vi "RDC-calculate_length.vi"(11 "Element map":map{dbl, T1}(c390)) -> (2 "L":dbl[](array[numeric]))   [LabVIEW 2020, in "RDC-Reflection_Data_Computation.lvlib"]
doc: "Takes an element map (frequency to data point) and returns an array of lengths L, one per frequency."
uses:
  RDC-Reflection_Data_Computation.lvlib
  Reflector/RFH-common_data_format_element.ctl
  Reflector/RFH-Reflection_File_Handler.lvlib
panel:
  out "Tau":dbl[](array[numeric])
  out "tau":dbl
  out "arctan(x)":dbl
  out "Theta":dbl
  out "l":dbl format="%#_6p"
  out "vp":dbl
  out "Beta":dbl
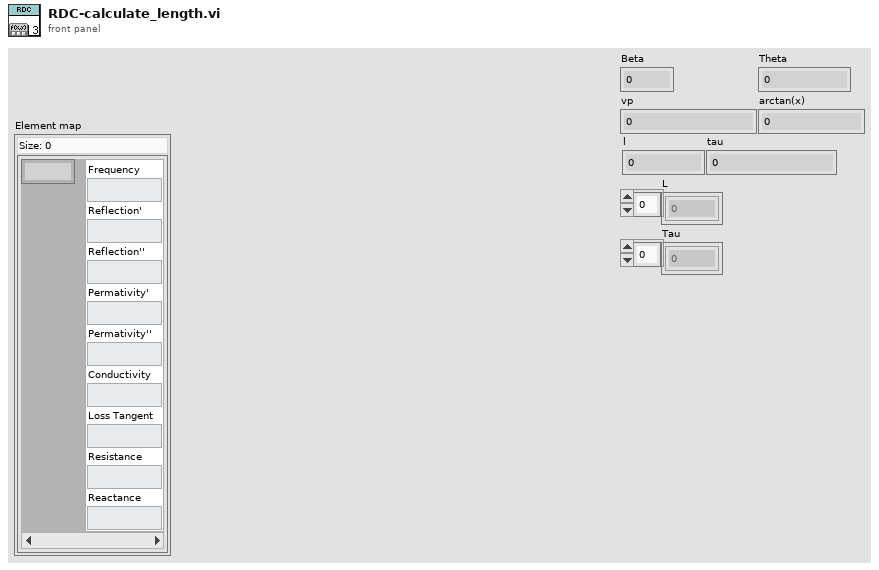
[diagram p1: front panel]
types:
  T1 = typedef "RFH-Reflection_File_Handler.lvlib/RFH-common_data_format_element.ctl" = cluster{"Frequency":dbl, "Reflection'":dbl, "Reflection''":dbl, "Permativity'":dbl, "Permativity''":dbl, "Conductivity":dbl, "Loss Tangent":dbl, "Resistance":dbl, "Reactance":dbl}
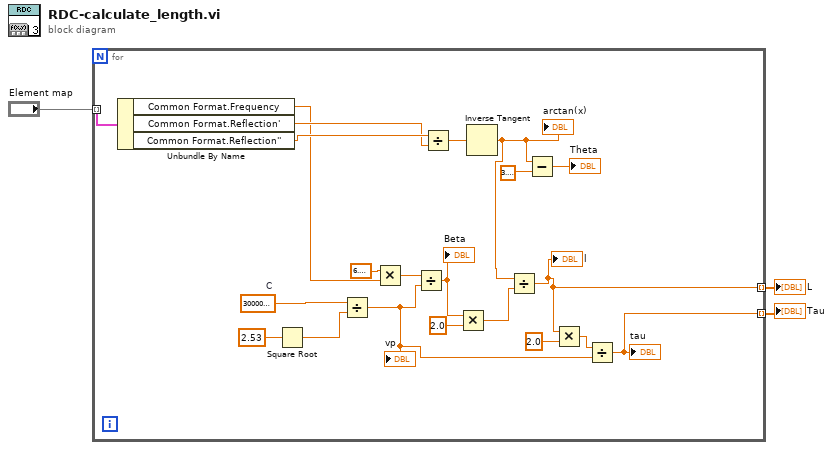
[diagram p0: block diagram]
diagram:
  n1 = for {
    tunnel: "Element map" -> [w24] mode=indexing
    tunnel: [w5] -> w2 mode=indexing
    tunnel: [w4] -> w1 mode=indexing
    w23 = 300000000.0  # C
    n2 = Unbundle By Name(w24) -> ("Common Format.Frequency"=w6:dbl, "Common Format.Reflection'"=w7:dbl, "Common Format.Reflection''"=w8:dbl)
    n3 = Square Root(x=2.53) -> (sqrt(x)=w21:dbl)
    n4 = Divide(x=w23, y=w21) -> (x/y=w9:dbl)
    "vp" <- w9
    n5 = Multiply(x=6.283185307179586, y=w6) -> (x*y=w19:dbl)
    n6 = Divide(x=w19, y=w9) -> (x/y=w18:dbl)
    "Beta" <- w18
    n7 = Divide(x=w8, y=w7) -> (x/y=w15:dbl)
    n8 = Multiply(x=w18, y=2.0) -> (x*y=w16:dbl)
    n9 = Inverse Tangent(1:w15) -> (0:w12:dbl)
    "arctan(x)" <- w12
    n10 = Divide(x=w12, y=w16) -> (x/y=w5:dbl)
    "l" <- w5
    n11 = Subtract(x=w12, y=3.141592653589793) -> (x-y=→"Theta":dbl)
    n12 = Multiply(x=w5, y=2.0) -> (x*y=w10:dbl)
    n13 = Divide(x=w10, y=w9) -> (x/y=w4:dbl)
    "tau" <- w4
  }
  "L" <- w2
  "Tau" <- w1
